vi "Remove_empty.vi"(11 "ARR_in":string[][](array[string])) -> (3 "ARR_out":string[][](array[string]))   [LabVIEW 2025, in "Procotol_class.lvclass"]
uses:
  Procotol_class.lvclass
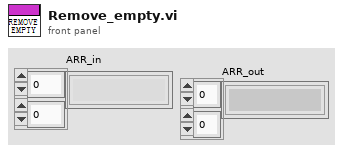
[diagram p1: front panel]
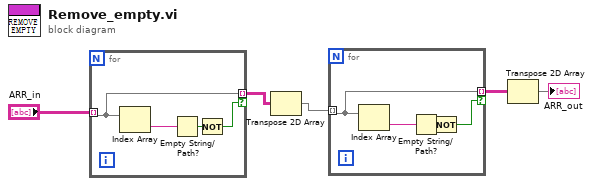
[diagram p0: block diagram]
diagram:
  n1 = for {
    tunnel: "ARR_in" -> [w8] mode=indexing
    tunnel: [w8] -> w4 mode=indexing if=w6
    n2 = Index Array(array=w8) -> (element=w9:string)  [unwired: 1 in]
    n3 = Empty String/Path?(string/path=w9) -> (empty?=w7:bool)
    n4 = Not(x=w7) -> (.not. x?=w6:bool)
  }
  n5 = Transpose 2D Array(2D array=w4) -> (transposed array=w3:string[][])
  n6 = for {
    tunnel: w3 -> [w12] mode=indexing
    tunnel: [w12] -> w2 mode=indexing if=w10
    n7 = Index Array(array=w12) -> (element=w13:string)  [unwired: 1 in]
    n8 = Empty String/Path?(string/path=w13) -> (empty?=w11:bool)
    n9 = Not(x=w11) -> (.not. x?=w10:bool)
  }
  n10 = Transpose 2D Array(2D array=w2) -> (transposed array=→"ARR_out":string[][])
